vi "Asylum_Driver_Plugin_IVCurve.vi"(4 "Abort Notifier":refnum<notifier>, 6 "Interpolation":dbl format="%#_13g", 7 "Writing Setpoint":dbl=0.1 format="%#_13g", 8 "error in (no error)":errorcluster, 9 "Offsets":cluster{"X":dbl, "Y":dbl}, 10 "Pattern Data":T2={"Name"="", "Litho"=[], "Set Resistance"=enum."1G ohm", "Meta"=variant}, 11 "Application":refnum<k7>) -> (0 "error out":errorcluster, 1 "Y":dbl[](array[numeric]), 2 "X":dbl[](array[numeric]), 3 "Application Out":refnum<k7>)   [LabVIEW 2019]
uses:
  <userlib>/LevyLab/Relay Box/Typedefs/Resistor--enum.ctl
  <userlib>/LevyLab/Relay Box/Relay-Box.lvclass
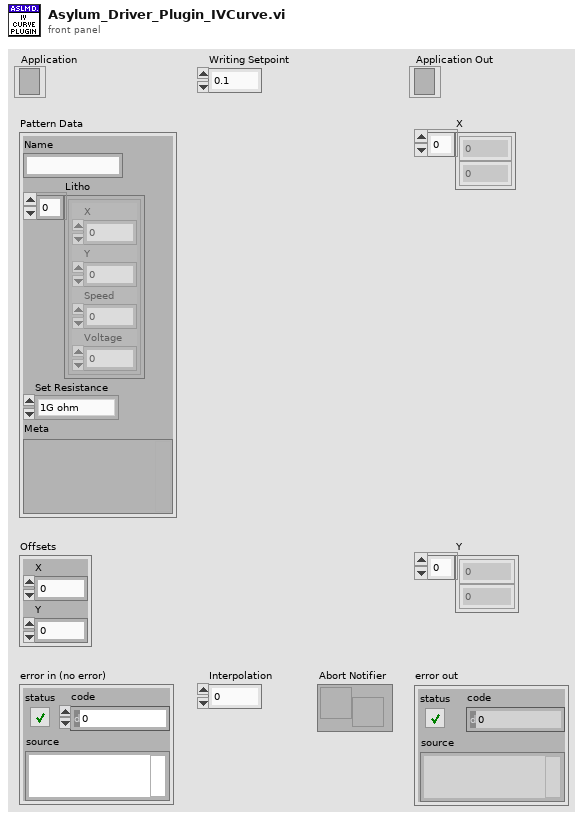
[diagram p1: front panel]
types:
  T1 = typedef "Relay-Box.lvclass/Resistor--enum.ctl" = enum16{"open", "discharge tip", "0 ohms", "100k ohm", "10M ohm", "1G ohm"}
  T2 = cluster{"Name":string, "Litho":cluster{"X":dbl, "Y":dbl, "Speed":dbl, "Voltage":dbl}[], "Set Resistance":T1, "Meta":variant}
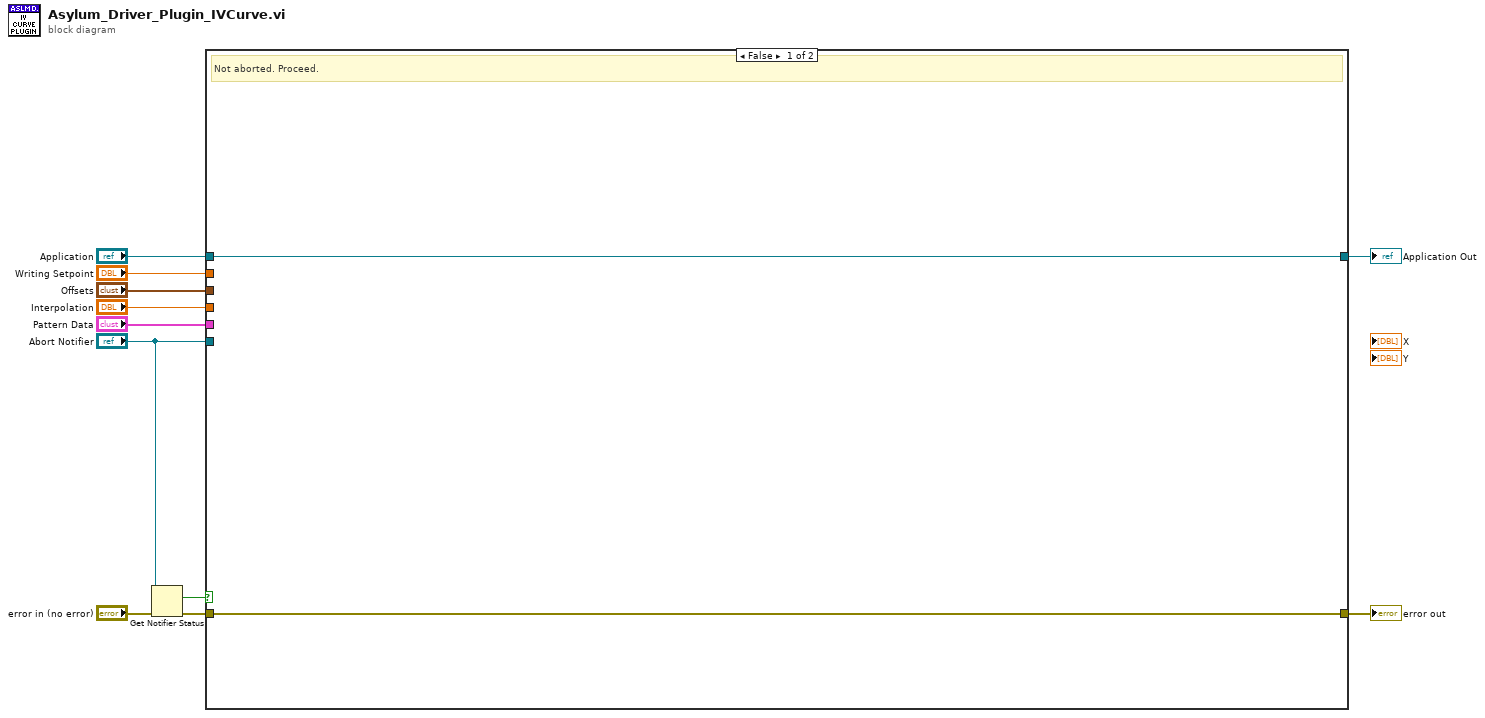
[diagram p0: block diagram]
diagram:
  n1 = Get Notifier Status(notifier="Abort Notifier", error in (no error)="error in (no error)") -> (current notification=w1:bool, error out=w3:errorcluster)  [unwired: 3 out]
  n2 = case shown="False" w1 {
    tunnel: [w12 w14] -> w11
    tunnel: "Application" -> [w13 w15]
    tunnel: "Writing Setpoint" -> [_ _]
    tunnel: "Offsets" -> [_ _]
    tunnel: "Interpolation" -> [_ _]
    tunnel: "Pattern Data" -> [_ _]
    tunnel: [w13 w15] -> w5
    tunnel: w3 -> [w12 w14]
    tunnel: "Abort Notifier" -> [_ _]
    frame False {
      # "Not aborted. Proceed."
    }
    frame True {
      # "Aborted. Do not run the plugin."
    }
  }
  "error out" <- w11
  "Application Out" <- w5
